vi "Spawn Child placeholder.vi"(11 "TEMPLATE Actor in":refnum<class "TEMPLATE Actor.lvclass">) -> (0 "Error out":errorcluster, 3 "TEMPLATE Actor out":refnum<class "TEMPLATE Actor.lvclass">)   [LabVIEW 2020, in "_Template.lvlib" / "Templates.lvlib" / "TEMPLATE jettl Actor.lvlib" / "TEMPLATE Actor.lvlib" / "TEMPLATE Actor.lvclass"]
uses:
  TEMPLATE Actor.lvclass
  C:/git/jettl/src/jettl/jettl/Actor/Actor.lvclass
  jettl/jettl/Actor/Actor.lvclass
  Child UIDs.ctl
  jettl/jettl/Base Attributes/Base Attributes/Base Attributes.lvclass/Base Attributes.ctl
  jettl/jettl/Unify.vi
  jettl/jettl/Base Attributes/Init Attributes.vi
  jettl/jettl/Insert Child Attributes.vi
  jettl/jettl/Check Parent Actor.vi
  jettl/jettl/Check UID Already Exists.vi
  jettl/jettl/Check UID Empty.vi
  jettl/jettl/Check Actors.vi
  jettl/jettl/Unify Iterator.vi
  jettl/jettl/Base Attributes/Base Attributes/Init Attributes.vi
  jettl/jettl/Find Child UIDs.vi
  jettl/jettl/Base Attributes/Base Attributes/Base Attributes.lvclass
  C:/git/jettl/src/jettl/jettl/Attributes/Attributes.lvclass
  jettl/jettl/Already In Stop--error.vi
  jettl/jettl/Not Concrete Actor--error.vi
  jettl/jettl/UID Empty--error.vi
  jettl/jettl/UID Already Exists--error.vi
  jettl/jettl/Async Actor.vi
  jettl/jettl/Transport/Transport.lvclass
  jettl/jettl/Msg/Msg.lvclass
  jettl/jettl/Attributes/Attributes.lvclass
  jettl/jettl/jettl.lvlib
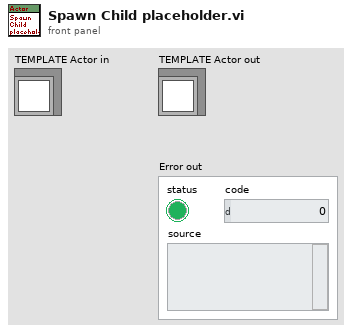
[diagram p1: front panel]
types:
  T1 = typedef "_Template.lvlib/Templates.lvlib/TEMPLATE jettl Actor.lvlib/TEMPLATE Actor.lvlib/TEMPLATE Actor.lvclass/Child UIDs.ctl" = enum16{"placeholder"}
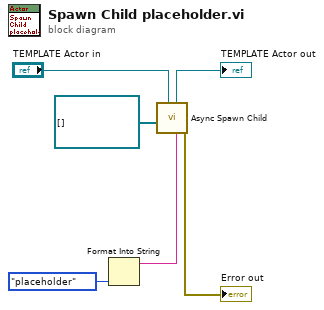
[diagram p0: block diagram]
diagram:
  n1 = Format Into String(Child_UIDs."placeholder" ("Child UIDs")) -> (resulting string=w4:string)  [unwired: 3 in, 1 out]
  n2 = call "Async Spawn Child.vi"("UID"=w4, "Actor in"="TEMPLATE Actor in", "Mid Actors"=refnum<class "Actor.lvclass">[] []) -> ("Error out"=→"Error out":errorcluster, "Actor out"=→"TEMPLATE Actor out":refnum<class "TEMPLATE Actor.lvclass">)  [unwired: 7 in]
